vi "Initialize 8 NEO Swerve Drive.vi"(11 "Drive PID Gains":T1) -> (0 "error out":errorcluster, 3 "(N-N-C-P) Swerve Motors":T2 {"Steer Scaling" format="%.2f"; "Drive Scaling" format="%.2f"; "Pod Locations (ft)"."Right Back" format="%.2f"; "Pod Locations (ft)"."Right Front" format="%.2f"; "Pod Locations (ft)"."Left Back" format="%.2f"; "Pod Locations (ft)"."Left Front" format="%.2f"})   [LabVIEW 2023]
doc: "Initialize motors (order is left-front, left-back, right-front, right-back) with PID coefficients. combine with"
uses:
  Type Definitions/Hardware/Swerve Drives/(NEO-NEO-ThroughBore-Pigeon2) Swerve.ctl
  Type Definitions/Data/Pod Positions.ctl
  Type Definitions/Hardware/Swerve Configs/NEO-NEO-ThroughBore-Pigeon2 Swerve Config.ctl
  <vilib>/REVLibDriver/REVLibDriver.lvlib
  <resource>/objmgr/REVSpark.rc
  <vilib>/REV Custom Controls/Spark Voltage Compensation.ctl
  <vilib>/REV Custom Controls/REVSparkRefnum.ctl
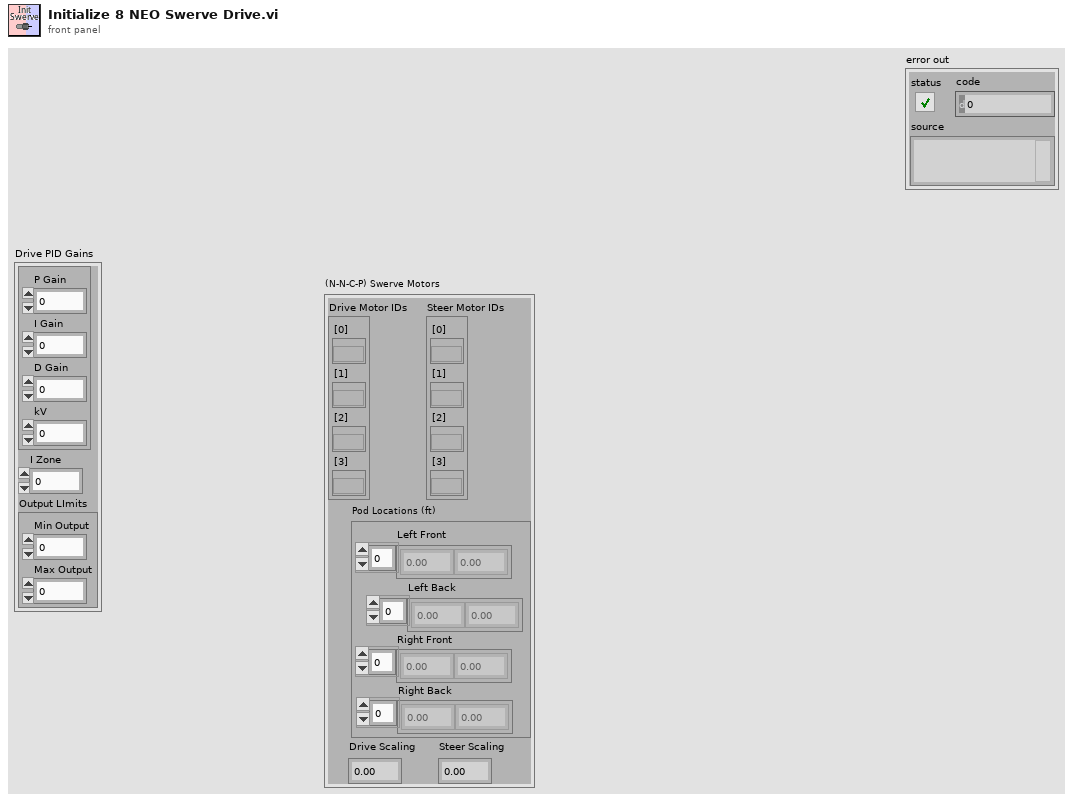
[diagram p1: front panel]
types:
  T1 = cluster{cluster{"P Gain":dbl, "I Gain":dbl, "D Gain":dbl, "kV":dbl}, "I Zone":dbl, "Output LImits":cluster{"Min Output":dbl, "Max Output":dbl}}
  T2 = typedef "(NEO-NEO-ThroughBore-Pigeon2) Swerve.ctl" = cluster{"Drive Motor IDs":cluster{"[0]":T3, "[1]":T3, "[2]":T3, "[3]":T3}, "Steer Motor IDs":cluster{"[0]":T3, "[1]":T3, "[2]":T3, "[3]":T3}, "Pod Locations (ft)":T4, "Drive Scaling":dbl, "Steer Scaling":dbl}
  T3 = typedef "REVLibDriver.lvlib/REVSparkRefnum.ctl" = refnum<k20>
  T4 = typedef "Pod Positions.ctl" = cluster{"Left Front":dbl[], "Left Back":dbl[], "Right Front":dbl[], "Right Back":dbl[]}
  T5 = typedef "NEO-NEO-ThroughBore-Pigeon2 Swerve Config.ctl" = cluster{"Bus ID":dbl, "Drive Motor CAN IDs":cluster{"LF CAN ID":dbl, "LB CAN ID":dbl, "RF CAN ID":dbl, "RB CAN ID":dbl}, "Steer Motor CAN IDs":cluster{"LF CAN ID":dbl, "LB CAN ID":dbl, "RF CAN ID":dbl, "RB CAN ID":dbl}, "Drive PID Gains":cluster{cluster{"P Gain":dbl, "I Gain":dbl, "D Gain":dbl, "kV":dbl}, "I Zone":dbl, "Output LImits":cluster{"Min Output":dbl, "Max Output":dbl}}, "Steer PID Gains":cluster{cluster{"P Gain":dbl, "I Gain":dbl, "D Gain":dbl, "kV":dbl}, "I Zone":dbl, "Output LImits":cluster{"Min Output":dbl, "Max Output":dbl}}, "Pod Locations (ft)":T4, "Inverted":cluster{"LF Inverted?":bool, "LFBInverted":bool, "RF Inverted":bool, "RB Inverted":bool}}
  T6 = cluster{"LF CAN ID":dbl, "LB CAN ID":dbl, "RF CAN ID":dbl, "RB CAN ID":dbl}
  T7 = typedef "REVLibDriver.lvlib/Spark Voltage Compensation.ctl" = cluster{"Mode":u32, "Nominal Voltage":dbl}
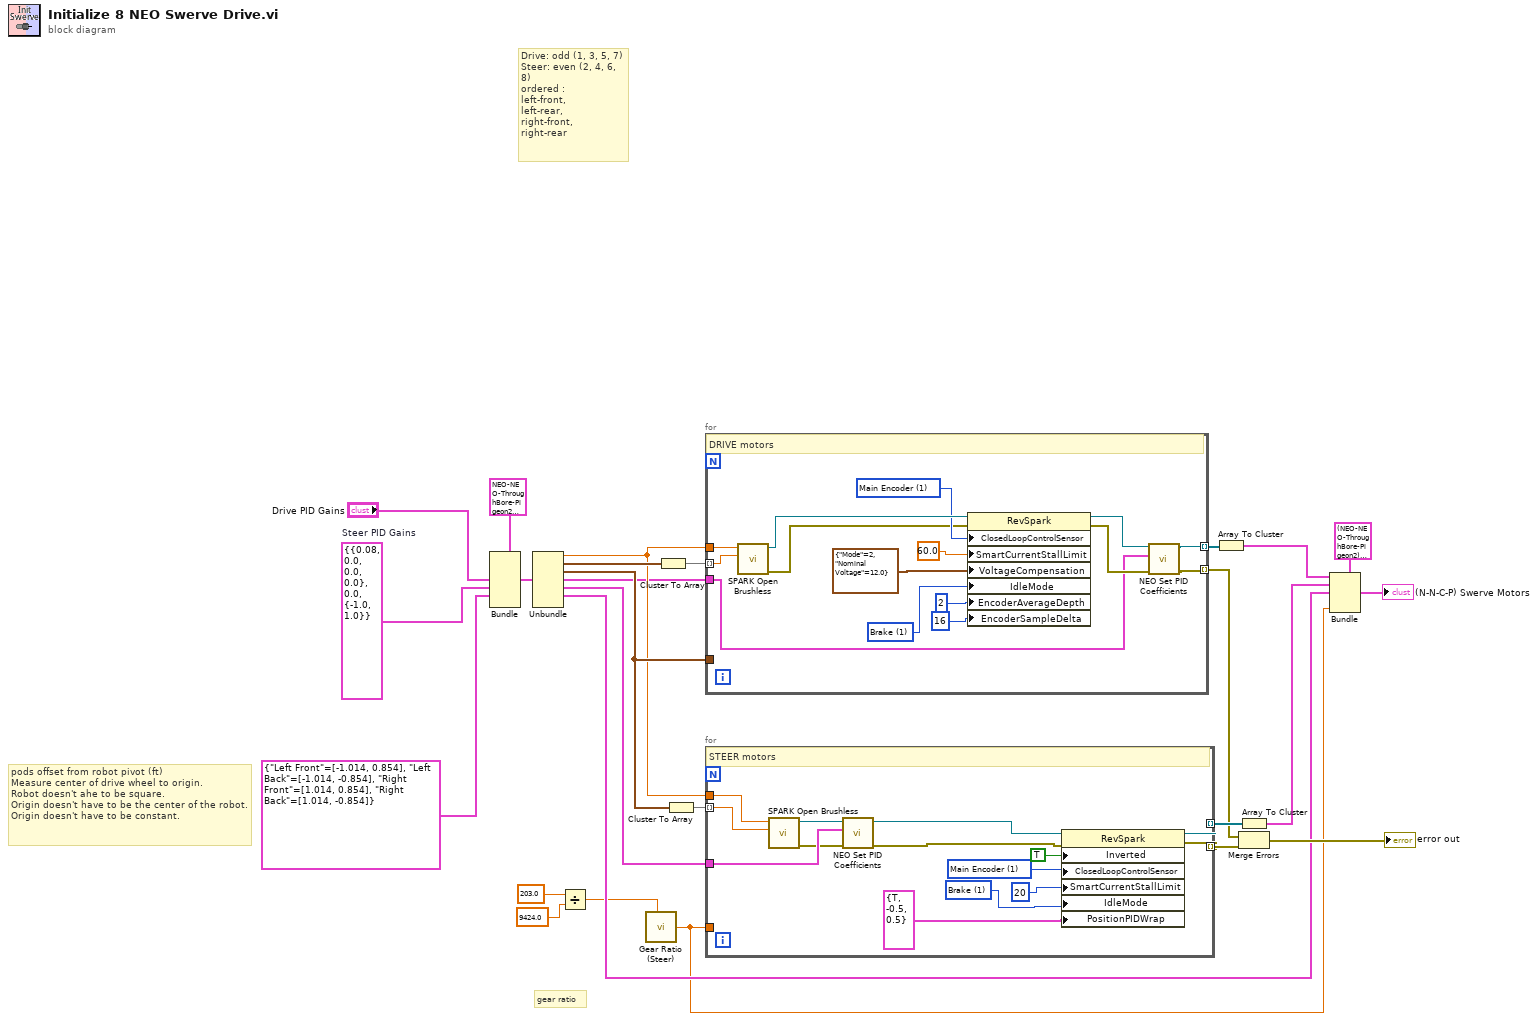
[diagram p0: block diagram]
diagram:
  w4 = T1 {{"P Gain"=0.08, "I Gain"=0.0, "D Gain"=0.0, "kV"=0.0}, "I Zone"=0.0, "Output LImits"={"Min Output"=-1.0, "Max Output"=1.0}}  # Steer PID Gains
  # "gear ratio"
  # "Drive: odd (1, 3, 5, 7)\nSteer: even (2, 4, 6, 8)\nordered :\nleft-front,\nleft-rear,\nright-front,\nright-rear"
  # "pods offset from robot pivot (ft)\nMeasure center of drive wheel to origin.\nRobot doesn't ahe to be square.\nOrigin doesn't have to be the center of the robot.\nOrigin doesn't have to be constant."
  n1 = Bundle(cluster=T5 {"Bus ID"=0.0, "Drive Motor CAN IDs"={"LF CAN ID"=1.0, "LB CAN ID"=3.0, "RF CAN ID"=5.0, "RB CAN ID"=7.0}, "Steer Motor CAN IDs"={"LF CAN ID"=2.0, "LB CAN ID"=4.0, "RF CAN ID"=6.0, "RB CAN ID"=8.0}, "Drive PID Gains"={{"P Gain"=0.12, "I Gain"=0.0, "D Gain"=0.0, "kV"=0.0}, "I Zone"=0.08, "Output LImits"={"Min Output"=-1.0, "Max Output"=1.0}}, "Steer PID Gains"={{"P Gain"=0.08, "I Gain"=0.0, "D Gain"=0.0, "kV"=0.0}, "I Zone"=0.0, "Output LImits"={"Min Output"=-1.0, "Max Output"=1.0}}, "Pod Locations (ft)"={"Left Front"=[], "Left Back"=[], "Right Front"=[], "Right Back"=[]}, "Inverted"={"LF Inverted?"=FALSE, "LFBInverted"=FALSE, "RF Inverted"=FALSE, "RB Inverted"=FALSE}} ("Swerve Config"), "Drive PID Gains"="Drive PID Gains", "Steer PID Gains"=w4, "Pod Locations (ft)"=T4 {"Left Front"=[-1.014, 0.854], "Left Back"=[-1.014, -0.854], "Right Front"=[1.014, 0.854], "Right Back"=[1.014, -0.854]} ("Radii (ft)")) -> (w24:T5)  [unwired: 4 in]
  n2 = Unbundle(w24) -> ("Bus ID"=w11:dbl, "Drive Motor CAN IDs"=w13:T6, "Steer Motor CAN IDs"=w12:T6, "Drive PID Gains"=w10:T1, "Steer PID Gains"=w9:T1, "Pod Locations (ft)"=w22:T4)  [unwired: 1 out]
  n3 = Divide(x=203.0, y=9424.0) -> (x/y=w1:dbl)
  n4 = call "Gear Ratio (Steer).vi"("Gear Ratio"=w1) -> ("Position Factor"=w6:dbl)  [unwired: 6 in, 1 out]
  n5 = Cluster To Array(cluster=w13) -> (array=w26:dbl[])
  n6 = Cluster To Array(cluster=w12) -> (array=w25:dbl[])
  n7 = for {
    tunnel: w26 -> [w41] mode=indexing
    tunnel: w12 -> [_]
    tunnel: [w28] -> w20 mode=indexing
    tunnel: [w27] -> w16 mode=indexing
    tunnel: w11 -> [w40]
    tunnel: w10 -> [w34]
    w31 = u32 1 items=["Coast", "Brake"] ("IdleMode")
    w38 = u32 1 items=["None", "Main Encoder", "Analog", "Alt Encoder", "Duty Cycle", "Detached Absolute", "Detached Relative"] ("ClosedLoopControlSensor")
    # "DRIVE motors"
    n8 = call <vilib>:"SPARK Open Brushless.vi"("deviceId"=w41, "busID"=w40) -> ("error out"=w36:errorcluster, "Spark refnum"=w39:T3)  [unwired: 8 in]
    n9 = property class="RevSpark"(reference=w39, error in=w36, "ClosedLoopControlSensor"=w38, "SmartCurrentStallLimit"=60.0 ("Primay Current Limit (80A)"), "VoltageCompensation"=T7 {"Mode"=2, "Nominal Voltage"=12.0}, "IdleMode"=w31, "EncoderAverageDepth"=u32 2, "EncoderSampleDelta"=u32 16) -> (reference out=w37:T3, error out=w35:errorcluster)
    n10 = call "NEO Set PID Coefficients.vi"("error in"=w35, "PID Gains"=w34, "Spark refnum"=w37) -> ("error out"=w27:errorcluster, "Spark refnum out"=w28:T3)  [unwired: 5 in]
  }
  n11 = for {
    tunnel: w25 -> [w54] mode=indexing
    tunnel: w9 -> [w55]
    tunnel: [w46] -> w18 mode=indexing
    tunnel: [w44] -> w17 mode=indexing
    tunnel: w11 -> [w53]
    tunnel: w6 -> [_]
    w50 = u32 1 items=["None", "Main Encoder", "Analog", "Alt Encoder", "Duty Cycle", "Detached Absolute", "Detached Relative"] ("ClosedLoopControlSensor")
    w48 = u32 1 items=["Coast", "Brake"] ("IdleMode")
    # "STEER motors"
    n12 = call <vilib>:"SPARK Open Brushless.vi"("deviceId"=w54, "busID"=w53) -> ("error out"=w51:errorcluster, "Spark refnum"=w52:T3)  [unwired: 8 in]
    n13 = call "NEO Set PID Coefficients.vi"("error in"=w51, "PID Gains"=w55, "Spark refnum"=w52) -> ("error out"=w45:errorcluster, "Spark refnum out"=w47:T3)  [unwired: 5 in]
    n14 = property class="RevSpark"(reference=w47, error in=w45, "Inverted"=TRUE ("Invert"), "ClosedLoopControlSensor"=w50, "SmartCurrentStallLimit"=u32 20, "IdleMode"=w48, "PositionPIDWrap"=cluster{"Enable":bool, "Min":sgl, "Max":sgl} {"Enable"=TRUE, "Min"=-0.5, "Max"=0.5}) -> (reference out=w46:T3, error out=w44:errorcluster)
  }
  n15 = Array To Cluster(array=w20) -> (cluster=w15:cluster{"[0]":T3, "[1]":T3, "[2]":T3, "[3]":T3})
  n16 = Array To Cluster(array=w18) -> (cluster=w19:cluster{"[0]":T3, "[1]":T3, "[2]":T3, "[3]":T3})
  n17 = Merge Errors(w16, w17) -> (→"error out":errorcluster)
  n18 = Bundle(cluster=T2 {"Drive Motor IDs"={"[0]"=refnum, "[1]"=refnum, "[2]"=refnum, "[3]"=refnum}, "Steer Motor IDs"={"[0]"=refnum, "[1]"=refnum, "[2]"=refnum, "[3]"=refnum}, "Pod Locations (ft)"={"Left Front"=[], "Left Back"=[], "Right Front"=[], "Right Back"=[]}, "Drive Scaling"=0.0, "Steer Scaling"=0.0} ("(N-N-C-P) Swerve Motors"), "Drive Motor IDs"=w15, "Steer Motor IDs"=w19, "Pod Locations (ft)"=w22, "Steer Scaling"=w6) -> (→"(N-N-C-P) Swerve Motors":T2)  [unwired: 1 in]
